vi "ZM-CI-handlePackage.vi"(8 "error in (no error)":errorcluster, 10 "package":refnum<class "ZM-PC-package.lvclass">, 11 "ZM-CM-communication_manager in":refnum<class "ZM-CM-communication_manager.lvclass">) -> (0 "error out":errorcluster, 3 "ZM-CM-communication_manager out":refnum<class "ZM-CM-communication_manager.lvclass">)   [LabVIEW 2020, in "ZM-CM-communication_manager.lvlib" / "ZM-CM-communication_manager.lvclass"]
doc: "Override of the interface method ZM-CI-package_handler:ZM-CI-handlePackage (public, dynamic dispatch), called by the Do.vi of ZM-CI-handlePackage Msg: Read protocol -> ZM-CP-publish(package) (dynamic dispatch) -> Write protocol; Read publishedCount -> +1 -> Write publishedCount. One error chain through every call; a publish error reaches Do.vi and so Handle Error."
uses:
  ZM-CM-communication_manager.lvclass
  common/ZM-PC-packages/ZM-PC-package/ZM-PC-package.lvclass
  ZM-CM-communication_manager.lvclass/ZM-CM-communication_manager.ctl
  protocol/ZM-CP-communication_protocol/ZM-CP-communication_protocol/ZM-CP-communication_protocol.lvclass
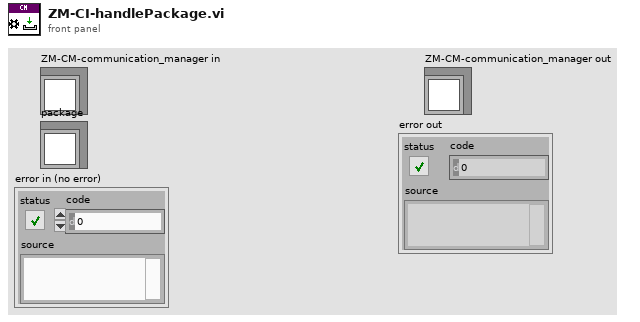
[diagram p1: front panel]
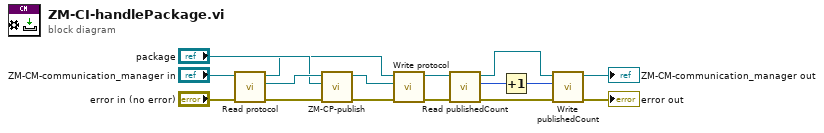
[diagram p0: block diagram]
diagram:
  n1 = call "Read protocol.vi"("error in (no error)"="error in (no error)", "ZM-CM-communication_manager in"="ZM-CM-communication_manager in") -> ("error out"=w12:errorcluster, "ZM-CP-communication_protocol.lvlib:ZM-CP-communication_protocol.lvclass"=w14:refnum<class "ZM-CP-communication_protocol.lvclass">, "ZM-CM-communication_manager out"=w10:refnum<class "ZM-CM-communication_manager.lvclass">)  [unwired: 7 in]
  n2 = call-dynamic "ZM-CP-publish.vi"("error in (no error)"=w12, "package"="package", "ZM-CP-communication_protocol in"=w14) -> ("error out"=w11:errorcluster, "ZM-CP-communication_protocol out"=w9:refnum<class "ZM-CP-communication_protocol.lvclass">)  [unwired: 7 in]
  n3 = call "Write protocol.vi"("error in (no error)"=w11, "ZM-CP-communication_protocol.lvlib:ZM-CP-communication_protocol.lvclass"=w9, "ZM-CM-communication_manager in"=w10) -> ("error out"=w8:errorcluster, "ZM-CM-communication_manager out"=w7:refnum<class "ZM-CM-communication_manager.lvclass">)  [unwired: 7 in]
  n4 = call "Read publishedCount.vi"("error in (no error)"=w8, "ZM-CM-communication_manager in"=w7) -> ("error out"=w5:errorcluster, "publishedCount"=w6:u32, "ZM-CM-communication_manager out"=w4:refnum<class "ZM-CM-communication_manager.lvclass">)  [unwired: 7 in]
  n5 = Increment(x=w6) -> (x+1=w3:u32)
  n6 = call "Write publishedCount.vi"("error in (no error)"=w5, "publishedCount"=w3, "ZM-CM-communication_manager in"=w4) -> ("error out"=→"error out":errorcluster, "ZM-CM-communication_manager out"=→"ZM-CM-communication_manager out":refnum<class "ZM-CM-communication_manager.lvclass">)  [unwired: 7 in]
